vi "MDPtr IsValidPtr.vi"(9 "error in (no error)":errorcluster, 10 "HexStrPtr":T1) -> (1 "Valid MDPtr?":bool, 2 "error out":errorcluster, 3 "HexStrPtr (dup)":T1)   [LabVIEW 2017, in "MDPtr.lvlib"]
uses:
  MDPtr.lvlib
  MDPtr TypeDef/MDPtr.ctl
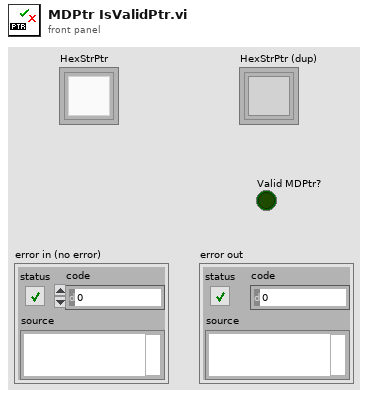
[diagram p1: front panel]
types:
  T1 = typedef "MDPtr.lvlib/MDPtr.ctl" = refnum<k1>
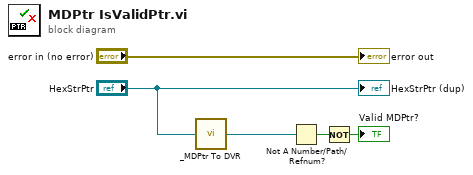
[diagram p0: block diagram]
diagram:
  n1 = call "_MDPtr To DVR.vi"("MDPtr"="HexStrPtr") -> ("MDPtr DVR"=w3:refnum<data-value>)
  n2 = Not A Number/Path/Refnum?(number/path/refnum=w3) -> (NaN/Path/Refnum?=w2:bool)
  n3 = Not(x=w2) -> (.not. x?=→"Valid MDPtr?":bool)
  "error out" <- "error in (no error)"
  "HexStrPtr (dup)" <- "HexStrPtr"
